vi "Tosca-Evaluate Sequence Expression.vi"(0 "Expr in":string, 9 "Nrand":i32=1, 11 "error in (no error)":errorcluster) -> (4 "Values":dbl[](array[numeric]), 15 "error out":errorcluster)   [LabVIEW 2020]
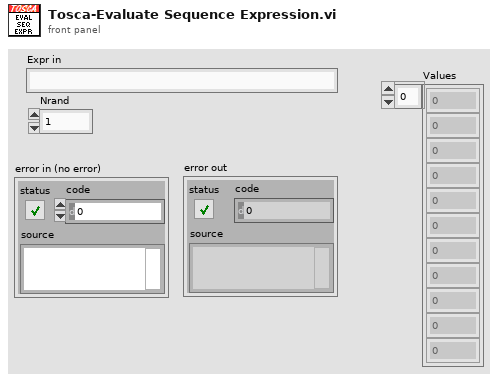
[diagram p1: front panel]
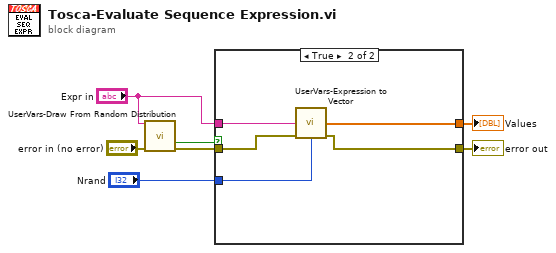
[diagram p0: block diagram]
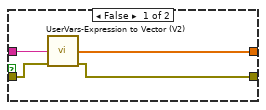
[diagram p2: hidden frame]
diagram:
  n1 = call "UserVars-Draw From Random Distribution.vi"("Expr in"="Expr in", "error in (no error)"="error in (no error)") -> ("found?"=w6:bool, "error out"=w5:errorcluster)  [unwired: 11 in, 1 out]
  n2 = case shown="True" w6 {
    tunnel: "Expr in" -> [w11 w15]
    tunnel: w5 -> [w10 w16]
    tunnel: [w9 w13] -> w4
    tunnel: [w8 w14] -> w3
    tunnel: "Nrand" -> [_ w12]
    frame False {
      n3 = call "UserVars-Expression to Vector (V2).vi"("Expr"=w11, "error in (no error)"=w10) -> ("Values"=w9:dbl[], "error out"=w8:errorcluster)  [unwired: 12 in]
    }
    frame True {
      n4 = call "UserVars-Expression to Vector.vi"("Expr"=w15, "error in (no error)"=w16, "Nrand"=w12) -> ("Values"=w13:dbl[], "error out"=w14:errorcluster)  [unwired: 11 in]
    }
  }
  "Values" <- w4
  "error out" <- w3
